vi "Create (From Structure).vi"(8 "error in (no error)":errorcluster, 10 "Structure":refnum<vi>) -> (0 "error out":errorcluster, 3 "JKI SM out":refnum<class "JKI SM.lvclass">)   [LabVIEW 2020, in "JKI State Machine API.lvlib" / "JKI SM.lvclass"]
uses:
  JKI SM.lvclass
  JKI SM.lvclass/JKI SM.ctl
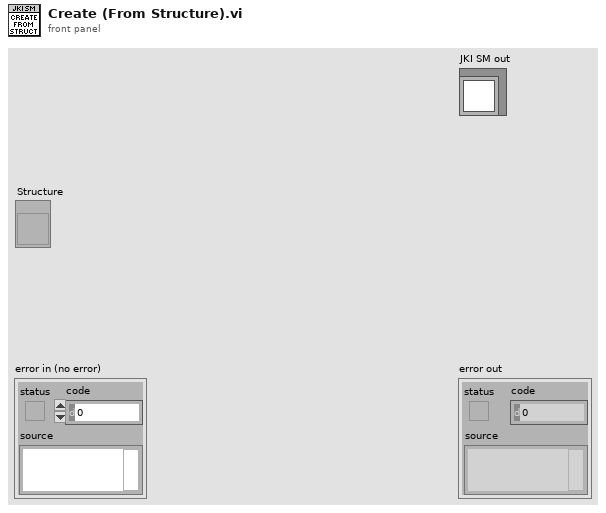
[diagram p1: front panel]
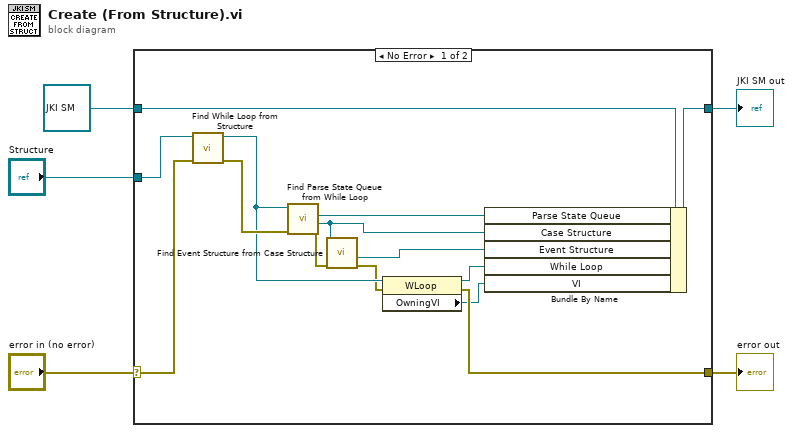
[diagram p0: block diagram]
diagram:
  n1 = case shown="No Error" "error in (no error)" {
    selector: "error in (no error)" -> [w12 w21]
    tunnel: [w7 w21] -> w1
    tunnel: [w18 w20] -> w3
    tunnel: refnum<class "JKI SM.lvclass"> refnum ("JKI SM") -> [w19 w20]
    tunnel: "Structure" -> [w13 _]
    frame No Error {
      n2 = call "Find While Loop from Structure.vi"("error in (no error)"=w12, "MultiFrameStructure in"=w13) -> ("error out"=w11:errorcluster, "WLoop Refnum"=w10:refnum<vi>)  [unwired: 8 in]
      n3 = call "Find Parse State Queue from While Loop.vi"("error in (no error)"=w11, "WhileLoop in"=w10) -> ("error out"=w14:errorcluster, "CaseStructure"=w16:refnum<vi>, "Parse State Queue"=w17:refnum<vi>)  [unwired: 7 in]
      n4 = call "Find Event Structure from Case Structure.vi"("error in (no error)"=w14, "CaseStructure"=w16) -> ("error out"=w8:errorcluster, "EvntStruct Refnum"=w15:refnum<vi>)  [unwired: 8 in]
      n5 = property class="WLoop"(reference=w10, error in=w8) -> (reference out=w9:refnum<vi>, error out=w7:errorcluster, "OwningVI"=w6:refnum<vi>)
      n6 = Bundle By Name(cluster=w19, "Parse State Queue"=w17, "Case Structure"=w16, "Event Structure"=w15, "While Loop"=w9, "VI"=w6) -> (w18:refnum<class "JKI SM.lvclass">)
    }
    frame Error {
    }
  }
  "error out" <- w1
  "JKI SM out" <- w3
